vi "Initialize Result.vi"(8 "error in (no error)":errorcluster, 10 "Count":i32, 11 "PQ Result":refnum<class "PQ Result.lvclass">) -> (0 "error out":errorcluster, 3 "PGJDPResult out":refnum<class "Result.lvclass">)   [LabVIEW 2020, in "ORM_pgsql_jdp.lvlib" / "Result.lvclass"]
uses:
  Result.lvclass
  <vilib>/JDP Science/PostgreSQL Library/Result/PQ Result.lvclass
  Result.lvclass/Result.ctl
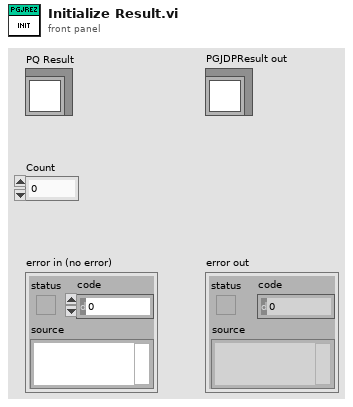
[diagram p1: front panel]
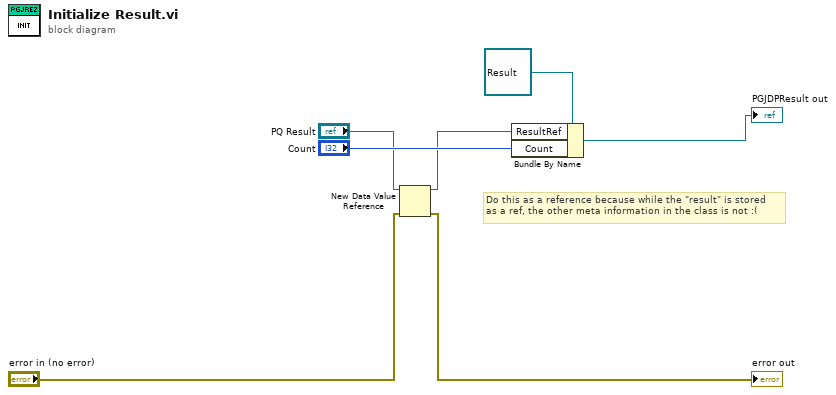
[diagram p0: block diagram]
diagram:
  # "Do this as a reference because while the \"result\" is stored\nas a ref, the other meta information in the class is not :("
  n1 = New Data Value Reference(data value="PQ Result", error in="error in (no error)") -> (data value reference=w5:refnum<data-value>, error out=→"error out":errorcluster)
  n2 = Bundle By Name(cluster=refnum<class "Result.lvclass"> refnum ("PGJDPResult out"), "ResultRef"=w5, "Count"="Count") -> (→"PGJDPResult out":refnum<class "Result.lvclass">)
